vi "Send Fundamental Frequency Response.vi"(8 "error in (no error)":errorcluster caption="에러 입력(에러 없음)", 9 "숫자형":dbl, 10 "id":string, 11 "Instrument Manager 입력":refnum<class "Instrument Manager.lvclass">) -> (0 "error out":errorcluster caption="에러 출력", 3 "Instrument Manager 출력":refnum<class "Instrument Manager.lvclass">)   [LabVIEW 2023, in "Instrument Manager.lvclass"]
uses:
  Instrument Manager.lvclass
  Fundamental Frequency Response.ctl
  Instrument Manager.lvclass/Instrument Manager.ctl
  Error Response.ctl
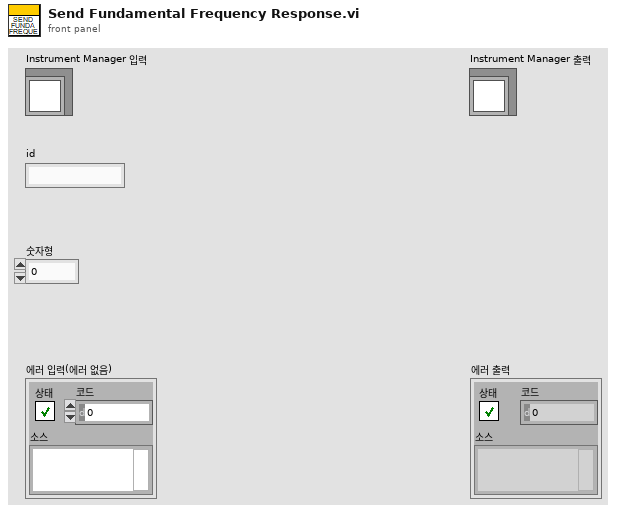
[diagram p1: front panel]
types:
  T1 = typedef "Instrument Manager.lvclass/Fundamental Frequency Response.ctl" = cluster{"type":string, "id":string, "status":string, "Result":cluster{"Fundamental Frequency":dbl}}
  T2 = cluster{"Reader Q":refnum<queue>, "Writer Q":refnum<queue>}
  T3 = typedef "Instrument Manager.lvclass/Error Response.ctl" = cluster{"type":string, "id":string, "status":string, "error out":errorcluster}
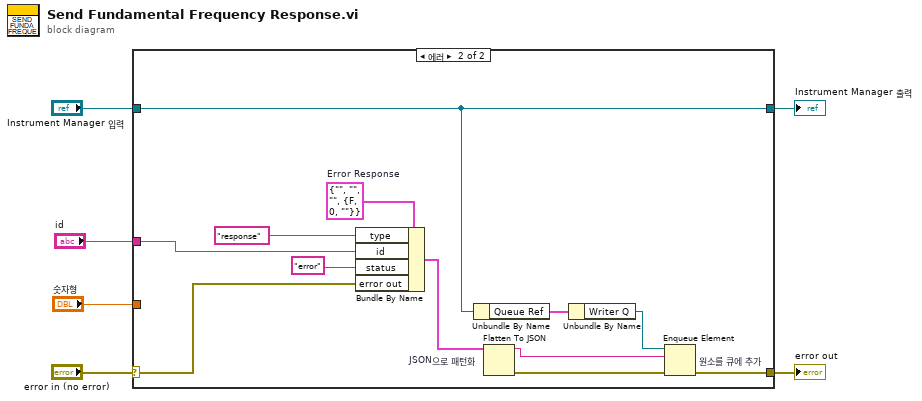
[diagram p0: block diagram]
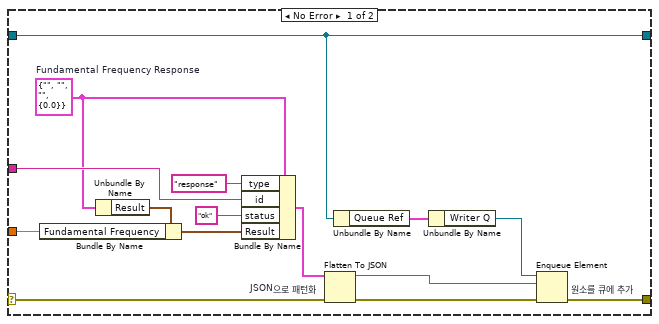
[diagram p2: hidden frame]
diagram:
  n1 = case shown="에러" "error in (no error)" {
    selector: "error in (no error)" -> [w9 w28]
    tunnel: [w8 w26] -> w5
    tunnel: [w7 w25] -> w3
    tunnel: "Instrument Manager 입력" -> [w7 w25]
    tunnel: "id" -> [w20 w22]
    tunnel: "숫자형" -> [w16 _]
    frame No Error {
      w18 = T1 {"type"="", "id"="", "status"="", "Result"={"Fundamental Frequency"=0.0}}  # Fundamental Frequency Response
      n2 = Unbundle By Name(w18) -> ("Result"=w17:cluster{"Fundamental Frequency":dbl})
      n3 = Bundle By Name(cluster=w17, "Fundamental Frequency"=w16) -> (w15:cluster{"Fundamental Frequency":dbl})
      n4 = Bundle By Name(cluster=w18, "type"="response", "id"=w20, "status"="ok", "Result"=w15) -> (w10:T1)
      n5 = Flatten To JSON "JSON으로 패턴화"(anything=w10, error in (no error)=w9) -> (JSON string=w11:string, 11:w13:errorcluster)  [unwired: 1 in]
      n6 = Unbundle By Name(w7) -> ("Queue Ref"=w14:T2)
      n7 = Unbundle By Name(w14) -> ("Writer Q"=w12:refnum<queue>)
      n8 = Enqueue Element "원소를 큐에 추가"(queue=w12, element=w11, error in (no error)=w13) -> (error out=w8:errorcluster)  [unwired: 1 in, 2 out]
    }
    frame Error {
      w33 = T3 {"type"="", "id"="", "status"="", "error out"={"status"=FALSE, "code"=0, "source"=""}}  # Error Response
      n9 = Bundle By Name(cluster=w33, "type"="response", "id"=w22, "status"="error", "error out"=w28) -> (w29:T3)
      n10 = Unbundle By Name(w25) -> ("Queue Ref"=w24:T2)
      n11 = Flatten To JSON "JSON으로 패턴화"(anything=w29) -> (JSON string=w32:string, 11:w27:errorcluster)  [unwired: 2 in]
      n12 = Unbundle By Name(w24) -> ("Writer Q"=w23:refnum<queue>)
      n13 = Enqueue Element "원소를 큐에 추가"(queue=w23, element=w32, error in (no error)=w27) -> (error out=w26:errorcluster)  [unwired: 1 in, 2 out]
    }
  }
  "error out" <- w5
  "Instrument Manager 출력" <- w3
